vi "Wire n terminal function.vi"(8 "error in (no error)":errorcluster, 9 "Sink Terminals":refnum<vi>[](array[refnum]), 10 "Source Terminals":refnum<vi>[](array[refnum]), 11 "Node In":refnum<vi>) -> (0 "error out":errorcluster, 2 "Function Output Terminals":refnum<vi>[](array[refnum]), 3 "Node Out":refnum<vi>)   [LabVIEW 2012, in "Scripting Tools.lvlib"]
doc: "Wires up a node with an arbitary number of terminals. The inputs to the node are connected to the terminals in the Source Terminals array, the ouptuts are connected to the terminals in the Sink Terminals array and are als returned in the Function Outouts array.\n\nSource Terminals and Sink Terminals need to be in the same order that the node orders its inputs and outputs."
uses:
  Scripting Tools.lvlib
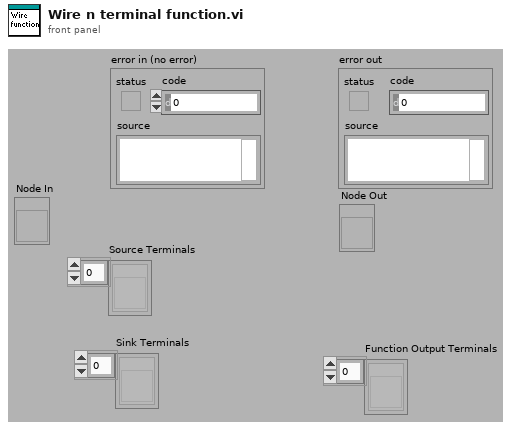
[diagram p1: front panel]
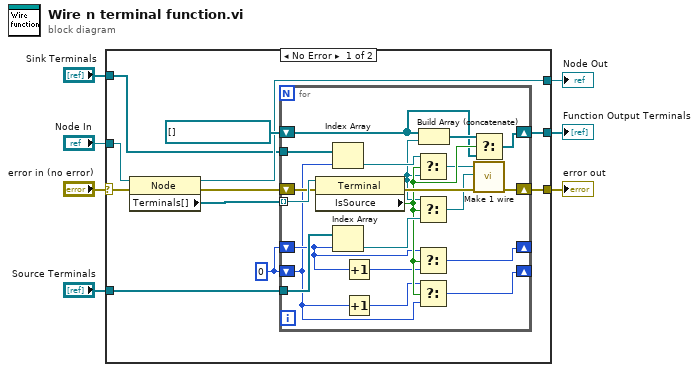
[diagram p0: block diagram]
diagram:
  n1 = case shown="No Error" "error in (no error)" {
    selector: "error in (no error)" -> [w8 w41]
    tunnel: [w14 _] -> w7
    tunnel: [w13 w41] -> w6
    tunnel: [w12 w40] -> w5
    tunnel: "Source Terminals" -> [w11 _]
    tunnel: "Sink Terminals" -> [w10 _]
    tunnel: "Node In" -> [w9 w40]
    frame No Error {
      w16 = 0
      n2 = property on="Property Node" class="Node"(reference=w9, error in=w8) -> (reference out=w12:refnum<vi>, error out=w18:errorcluster, "Terminals[]"=w17:refnum<vi>[])
      n3 = for {
        shift-right: [w21] -> w13
        shift-left: w18 -> [w38]
        tunnel: w17 -> [w39] mode=indexing
        shift-right: [w35] -> _
        shift-left: w16 -> [w24]
        shift-right: [w34] -> _
        shift-left: w16 -> [w22]
        shift-right: [w30] -> w14
        shift-left: refnum<vi>[] [] -> [w28]
        tunnel: w11 -> [w27]
        tunnel: w10 -> [w26]
        n4 = property on="Property Node" class="Terminal"(reference=w39, error in=w38) -> (reference out=w31:refnum<vi>, error out=w33:errorcluster, "IsSource"=w32:bool)
        n5 = Index Array(array=w26, index=w22) -> (element=w36:refnum<vi>)
        n6 = Index Array(array=w27, index=w24) -> (element=w37:refnum<vi>)
        n7 = Increment(x=w24) -> (x+1=w25:i32)
        n8 = Increment(x=w22) -> (x+1=w23:i32)
        n9 = Select(t=w36, s=w32, f=w31) -> (s? t:f=w20:refnum<vi>)
        n10 = Select(t=w31, s=w32, f=w37) -> (s? t:f=w19:refnum<vi>)
        n11 = Select(t=w24, s=w32, f=w25) -> (s? t:f=w35:i32)
        n12 = Select(t=w23, s=w32, f=w22) -> (s? t:f=w34:i32)
        n13 = Build Array (concatenate)(w28, w31) -> (w29:refnum<vi>[])
        n14 = Select(t=w29, s=w32, f=w28) -> (s? t:f=w30:refnum<vi>[])
        n15 = call "Make 1 wire.vi"("error in"=w33, "Wire Terminal 2"=w19, "Wire Terminal 1"=w20) -> ("error out"=w21:errorcluster)  [unwired: 8 out]
      }
    }
    frame Error {
    }
  }
  "Function Output Terminals" <- w7
  "error out" <- w6
  "Node Out" <- w5
